vi "Format Battery Description.vi"(0 "Chemistry":T2(ring), 5 "Measurement":T1, 7 "Alkaline Charge (%)":dbl, 9 "Ni-MH Charge (%)":dbl, 11 "error in":errorcluster) -> (4 "Description":string, 15 "error out":errorcluster)   [LabVIEW 2026]
doc: "Builds the one-line human-readable result of Classify Battery.vi: chemistry, approximate charge and the measured values, e.g. Alkaline, ~62 % (OCV 1.462 V, IR 0.31 Ohm). Li-ion 1.5V (BMS) reports its OCV and ripple instead of a charge; the ambiguous Alkaline or Ni-MH case reports the lower estimate and names both. NaN values print as n/a. Pure function: error in is passed to error out."
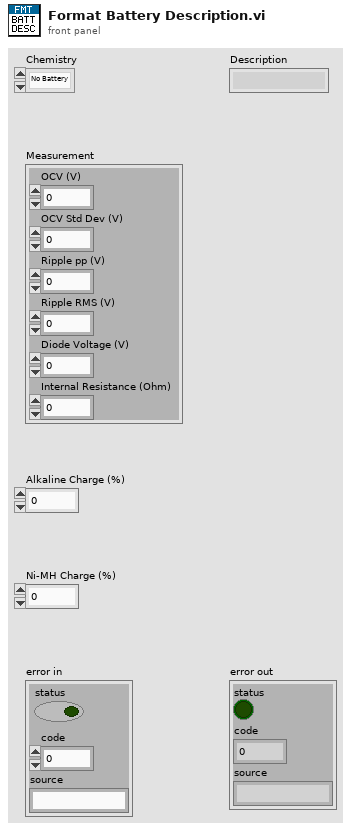
[diagram p1: front panel]
types:
  T1 = cluster{"OCV (V)":dbl, "OCV Std Dev (V)":dbl, "Ripple pp (V)":dbl, "Ripple RMS (V)":dbl, "Diode Voltage (V)":dbl, "Internal Resistance (Ohm)":dbl}
  T2 = enum16{"No Battery", "Reversed Polarity", "Alkaline", "Ni-MH", "Alkaline or Ni-MH", "Li-ion 1.5V (BMS)", "Depleted", "Unknown"}
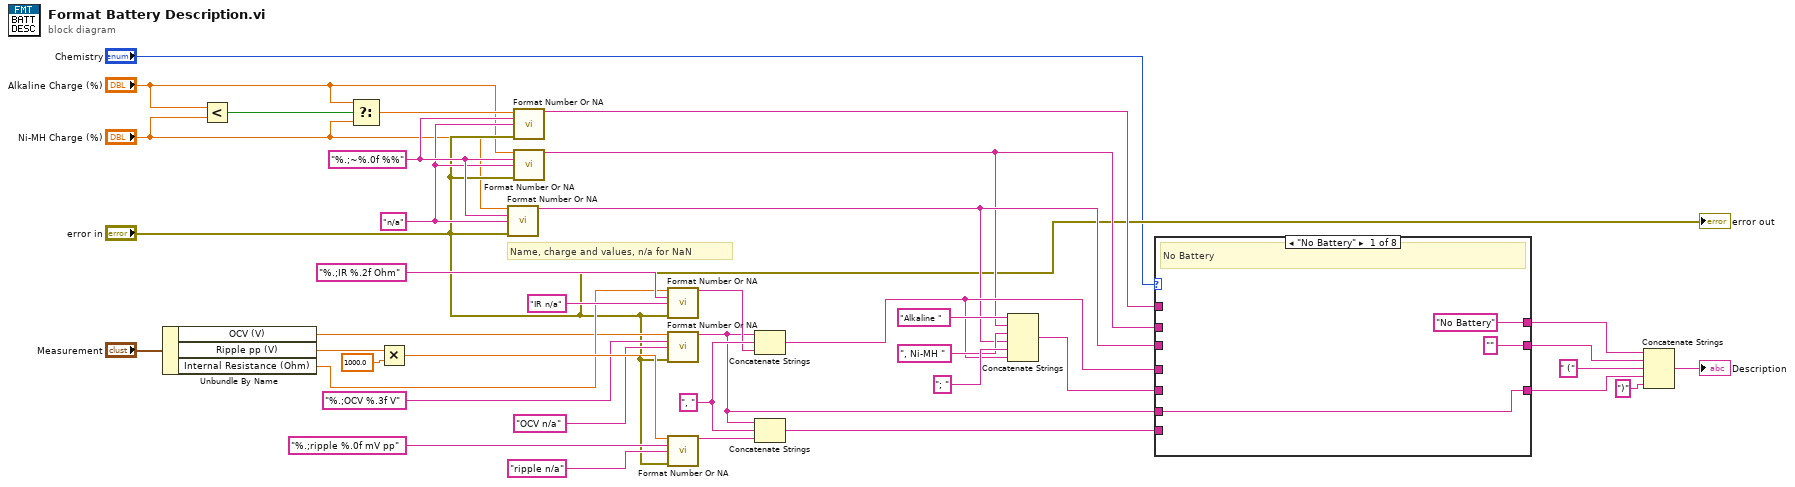
[diagram p0: block diagram]
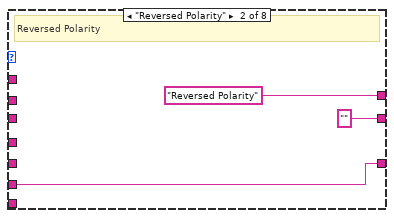
[diagram p2: hidden frame]
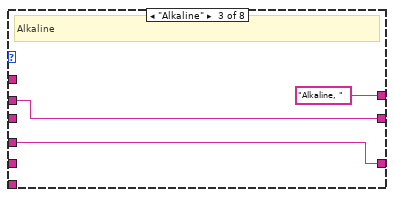
[diagram p3: hidden frame]
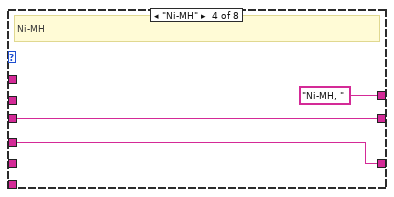
[diagram p4: hidden frame]
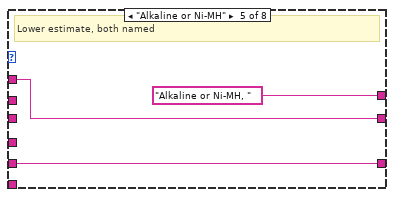
[diagram p5: hidden frame]
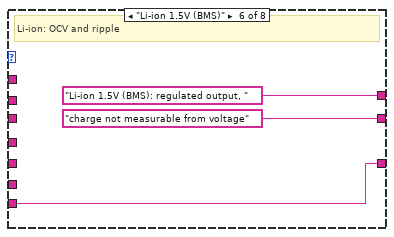
[diagram p6: hidden frame]
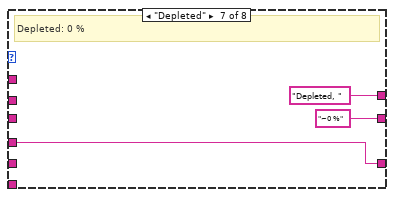
[diagram p7: hidden frame]
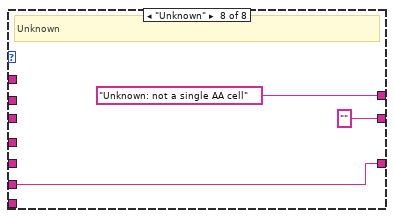
[diagram p8: hidden frame]
diagram:
  w27 = ", " ("separator")
  w12 = "%.;~%.0f %%" ("charge format")
  w11 = "n/a" ("n/a")
  # "Name, charge and values, n/a for NaN"
  n1 = Unbundle By Name("Measurement") -> ("OCV (V)"=w6:dbl, "Ripple pp (V)"=w7:dbl, "Internal Resistance (Ohm)"=w8:dbl)
  n2 = Less?(x="Alkaline Charge (%)", y="Ni-MH Charge (%)") -> (x < y?=w9:bool)
  n3 = Select(t="Alkaline Charge (%)", s=w9, f="Ni-MH Charge (%)") -> (s? t:f=w10:dbl)
  n4 = Multiply(x=w7, y=1000.0 ("mV per V")) -> (x*y=w23:dbl)
  n5 = call "Format Number Or NA.vi"("Value"="Ni-MH Charge (%)", "Format"=w12, "NaN Text"=w11, "error in"="error in") -> ("Text"=w14:string)  [unwired: 10 in, 1 out]
  n6 = call "Format Number Or NA.vi"("Value"=w10, "Format"=w12, "NaN Text"=w11, "error in"="error in") -> ("Text"=w15:string)  [unwired: 10 in, 1 out]
  n7 = call "Format Number Or NA.vi"("Value"="Alkaline Charge (%)", "Format"=w12, "NaN Text"=w11, "error in"="error in") -> ("Text"=w13:string)  [unwired: 10 in, 1 out]
  n8 = call "Format Number Or NA.vi"("Value"=w8, "Format"="%.;IR %.2f Ohm" ("IR format"), "NaN Text"="IR n/a" ("IR n/a"), "error in"="error in") -> ("Text"=w21:string)  [unwired: 10 in, 1 out]
  n9 = call "Format Number Or NA.vi"("Value"=w6, "Format"="%.;OCV %.3f V" ("OCV format"), "NaN Text"="OCV n/a" ("OCV n/a"), "error in"="error in") -> ("Text"=w18:string)  [unwired: 10 in, 1 out]
  n10 = call "Format Number Or NA.vi"("Value"=w23, "Format"="%.;ripple %.0f mV pp" ("ripple format"), "NaN Text"="ripple n/a" ("ripple n/a"), "error in"="error in") -> ("Text"=w26:string)  [unwired: 10 in, 1 out]
  n11 = Concatenate Strings(w18, w27, w21) -> (w28:string)
  n12 = Concatenate Strings(w18, w27, w26) -> (w29:string)
  n13 = Concatenate Strings("Alkaline " ("alkaline"), w13, ", Ni-MH " ("ni-mh"), w14, "; " ("semicolon"), w28) -> (w33:string)
  n14 = case shown="\"No Battery\"" "Chemistry" {
    tunnel: ["No Battery" ("name") "Reversed Polarity" ("name") "Alkaline, " ("name") "Ni-MH, " ("name") "Alkaline or Ni-MH, " ("name") "Li-ion 1.5V (BMS): regulated output, " ("name") "Depleted, " ("name") "Unknown: not a single AA cell" ("name")] -> w34
    tunnel: ["" ("charge text") "" ("charge text") w46 w49 w52 "charge not measurable from voltage" ("charge text") "~0 %" ("charge text") "" ("charge text")] -> w35
    tunnel: w13 -> [_ _ w46 _ _ _ _ _]
    tunnel: w14 -> [_ _ _ w49 _ _ _ _]
    tunnel: w18 -> [w40 w43 _ _ _ _ _ w61]
    tunnel: w15 -> [_ _ _ _ w52 _ _ _]
    tunnel: w28 -> [_ _ w47 w50 _ _ w58 _]
    tunnel: [w40 w43 w47 w50 w53 w55 w58 w61] -> w36
    tunnel: w29 -> [_ _ _ _ _ w55 _ _]
    tunnel: w33 -> [_ _ _ _ w53 _ _ _]
    frame "No Battery" {
      # "No Battery"
    }
    frame "Reversed Polarity" {
      # "Reversed Polarity"
    }
    frame "Alkaline" {
      # "Alkaline"
    }
    frame "Ni-MH" {
      # "Ni-MH"
    }
    frame "Alkaline or Ni-MH" {
      # "Lower estimate, both named"
    }
    frame "Li-ion 1.5V (BMS)" {
      # "Li-ion: OCV and ripple"
    }
    frame "Depleted" {
      # "Depleted: 0 %"
    }
    frame "Unknown" {
      # "Unknown"
    }
  }
  n15 = Concatenate Strings(w34, w35, " (" ("open"), w36, ")" ("close")) -> (→"Description":string)
  "error out" <- "error in"
